vi "ATE_CommCheck.vi"() -> ()   [LabVIEW 2026]
uses:
  <vilib>/NI/Modbus Library/API/Modbus API.lvclass/Modbus API.ctl
  <vilib>/NI/Modbus Library/Transmission Data Unit/Transmission Data Unit.lvclass/Transmission Data Unit.ctl
  <vilib>/NI/Modbus Library/Transmission Data Unit/Write Unit ID.vi
  <vilib>/NI/Modbus Library/API/Read Transmission Data Unit.vi
  <vilib>/NI/Modbus Library/API/Write Transmission Data Unit.vi
  <vilib>/NI/Modbus Library/API/Master/Modbus Master.lvclass
  C:/Program Files (x86)/National Instruments/LabVIEW 2026/vi.lib/NI/Modbus Library/API/Modbus API.lvclass
  <vilib>/NI/Modbus Library/API/Wrapper/Create TCP Master.vi
  <vilib>/NI/Modbus Library/API/Wrapper/API Main.lvlib
panel:
  out "쓰기 후 레지스터":u16[](array[numeric])
  out "쓰기 전 레지스터":u16[](array[numeric])
  out "error out":errorcluster
  out "처리 메시지":string
  out "응답 ID 쓰기 허가":bool
  in  "쓰기값":u16
  in  "동작":enum16{"읽기만", "시험 값 쓰기", "응답 ID 쓰기"}(ring)
  in  "Unit ID":u8
  in  "Port":u16
  in  "Server IP":string
  # "0 ATE_LINK_TEST\n1 ATE_REQUEST\n2 ATE_REQUEST_ID\n3 ATE_RESULT\n4 ATE_RESPONSE_ID\n5 ATE_DONE\n6 TEST_RESULT_LATCH\n7 SEQ_STATE\n8 ALARM_CODE"
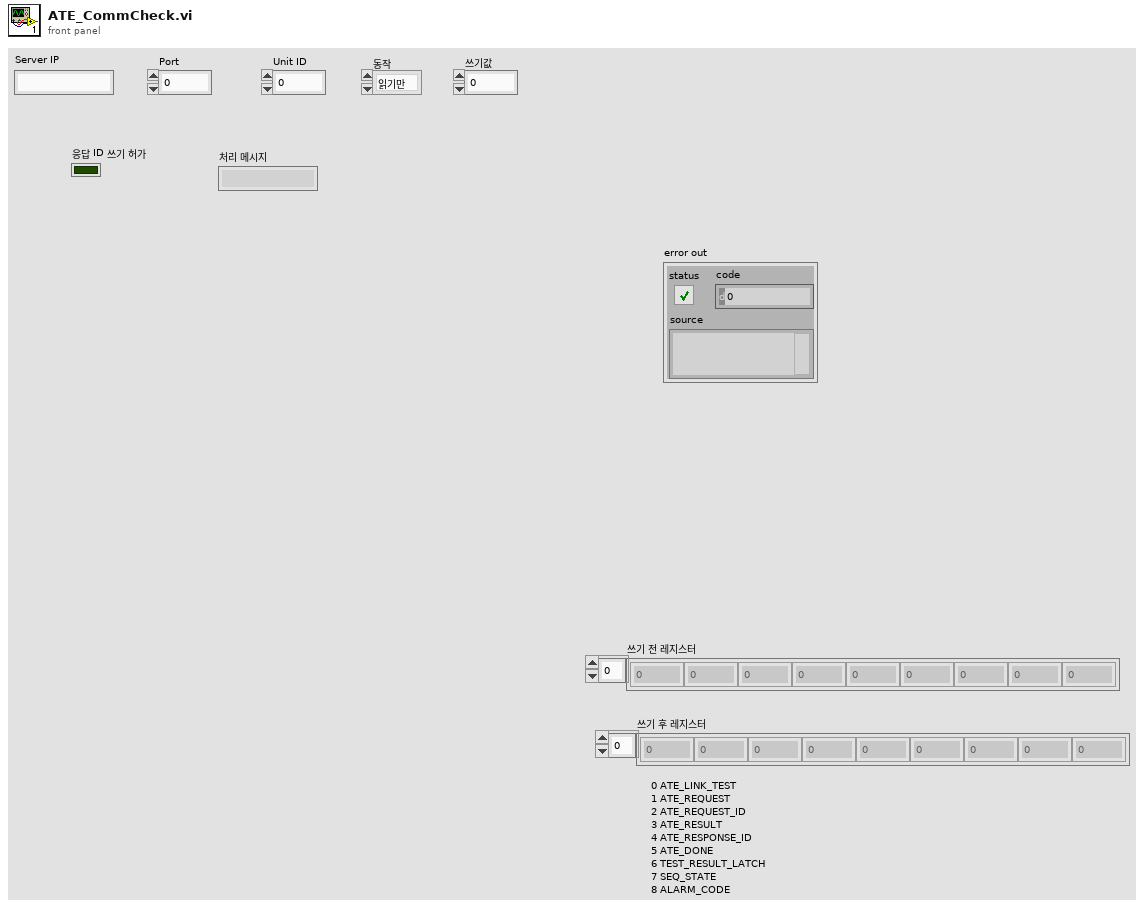
[diagram p1: front panel]
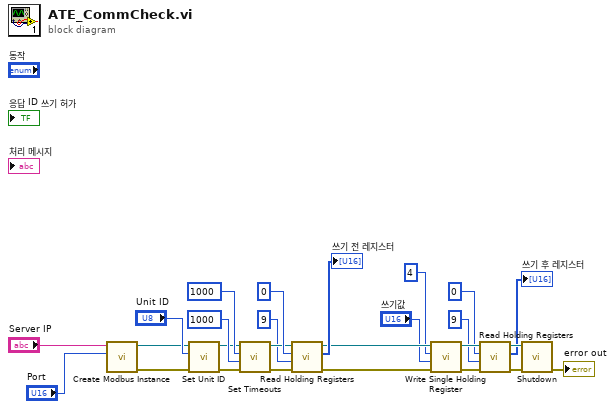
[diagram p0: block diagram]
diagram:
  n1 = call-poly <vilib>:"Create Modbus Instance.vi"("port (502)"="Port", "address"="Server IP") -> ("error out"=w19:errorcluster, "TCP master instance"=w20:refnum<class "Modbus Master.lvclass">)  [unwired: 8 in]
  n2 = call <vilib>:"Set Unit ID.vi"("error in"=w19, "unit ID"="Unit ID", "Modbus master in"=w20) -> ("error out"=w16:errorcluster, "Modbus master out"=w18:refnum<class "Modbus Master.lvclass">)  [unwired: 7 in]
  n3 = call <vilib>:"Set Timeouts.vi"("error in"=w16, "write operation timeout"=1000, "read operation timeout"=1000, "Modbus master in"=w18) -> ("error out"=w15:errorcluster, "Modbus master out"=w17:refnum<class "Modbus Master.lvclass">)  [unwired: 6 in]
  n4 = call-dynamic "Read Holding Registers.vi"("error in"=w15, "number of inputs"=u16 9, "starting address"=u16 0, "Modbus master in"=w17) -> ("error out"=w9:errorcluster, "register values"=→"쓰기 전 레지스터":u16[], "Modbus master out"=w11:refnum<class "Modbus Master.lvclass">)  [unwired: 5 in]
  n5 = call-dynamic "Write Single Holding Register.vi"("error in"=w9, "register to write"="쓰기값", "address"=u16 4, "Modbus master in"=w11) -> ("error out"=w8:errorcluster, "Modbus master out"=w10:refnum<class "Modbus Master.lvclass">)  [unwired: 6 in]
  n6 = call-dynamic "Read Holding Registers.vi"("error in"=w8, "number of inputs"=u16 9, "starting address"=u16 0, "Modbus master in"=w10) -> ("error out"=w7:errorcluster, "register values"=→"쓰기 후 레지스터":u16[], "Modbus master out"=w6:refnum<class "Modbus Master.lvclass">)  [unwired: 5 in]
  n7 = call-dynamic "Shutdown.vi"("error in"=w7, "Modbus master in"=w6) -> ("error out"=→"error out":errorcluster)  [unwired: 9 in]
